vi "Save Packets.vi"(5 "Save Format":u16, 6 "Headers":string[](array[string]), 7 "Path":path, 8 "error in":errorcluster, 9 "SAVE TO CSV":refnum<vi>, 10 "Packets":refnum<vi>, 11 "Interface Name String":string) -> (0 "error out":errorcluster, 3 "Status Message":string)   [LabVIEW 2025, in "Automotive Ethernet Bus Monitor UI.lvlib"]
doc: "Save the current Package Table to a file."
uses:
  Automotive Ethernet Bus Monitor UI.lvlib
  <vilib>/Utility/file.llb/Write Delimited Spreadsheet (string).vi
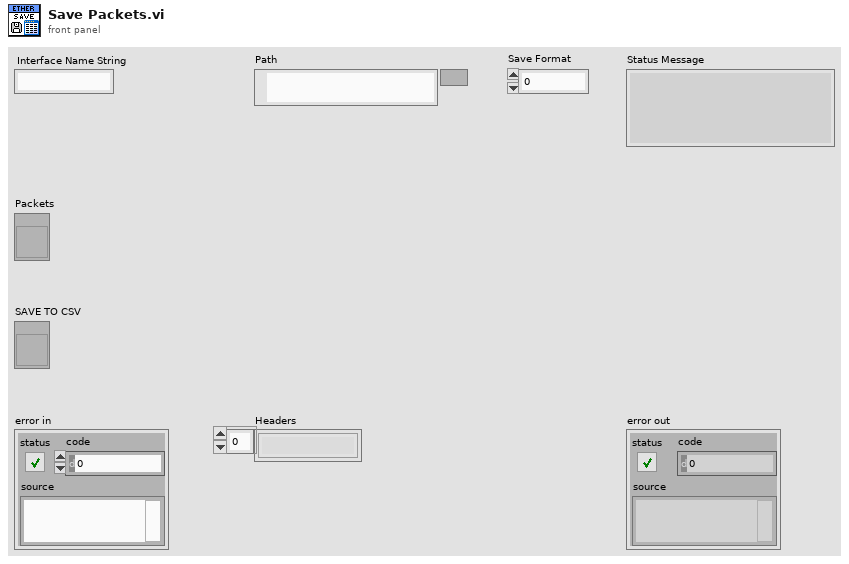
[diagram p1: front panel]
types:
  T1 = enum16{"open", "open or create", "create or replace", "create", "open (read-only)"}
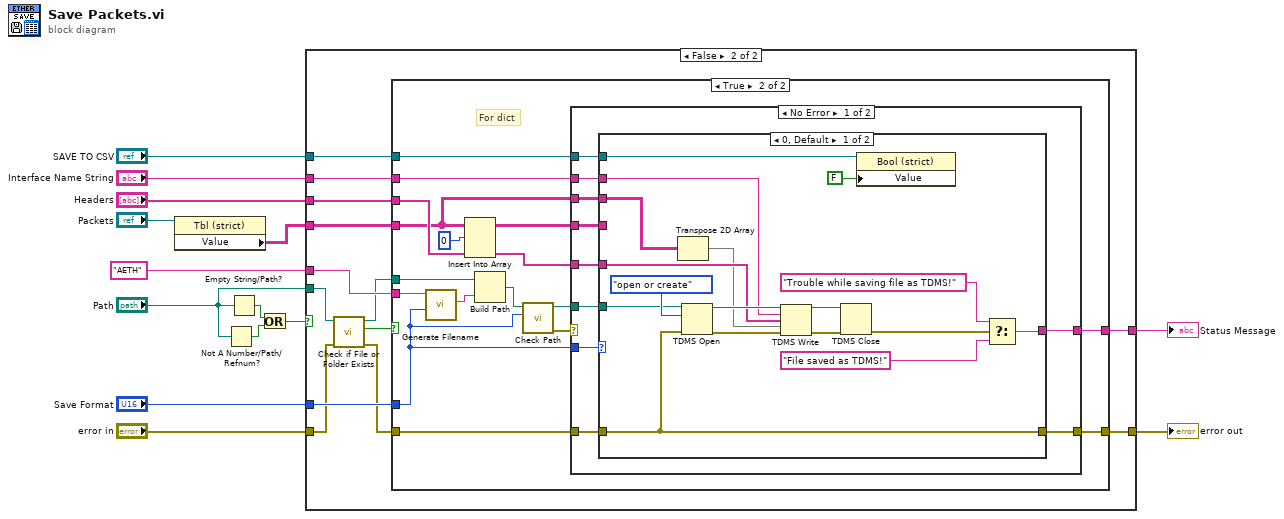
[diagram p0: block diagram]
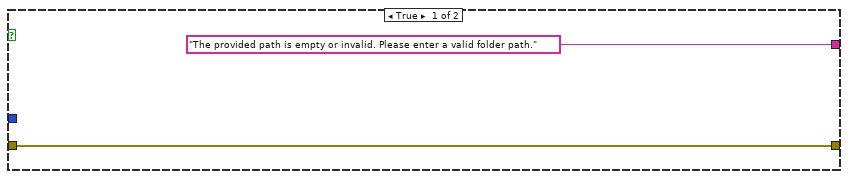
[diagram p2: hidden frame]
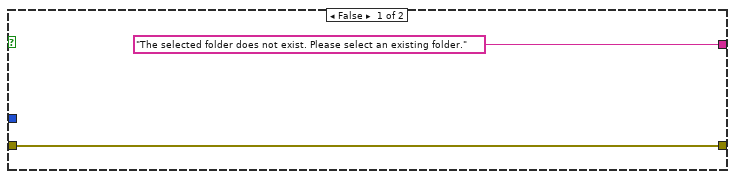
[diagram p3: hidden frame]
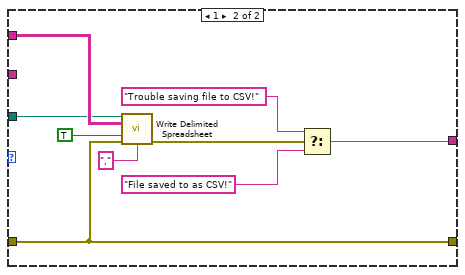
[diagram p4: hidden frame]
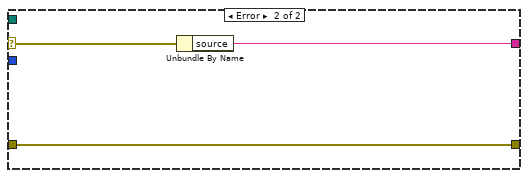
[diagram p5: hidden frame]
diagram:
  n1 = property class="Tbl (strict)"(reference="Packets") -> ("Value"=w5:string[][])  [unwired: 1 in, 2 out]
  n2 = Not A Number/Path/Refnum?(number/path/refnum="Path") -> (NaN/Path/Refnum?=w13:bool)
  n3 = Empty String/Path?(string/path="Path") -> (empty?=w12:bool)
  n4 = Or(x=w12, y=w13) -> (x .or. y?=w14:bool)
  n5 = case shown="False" w14 {
    tunnel: [w15 w29] -> w7
    tunnel: "Headers" -> [_ w28]
    tunnel: w5 -> [_ w27]
    tunnel: "error in" -> [w15 w19]
    tunnel: "Save Format" -> [_ w25]
    tunnel: "AETH" ("bustype in") -> [_ w24]
    tunnel: "Path" -> [_ w23]
    tunnel: ["The provided path is empty or invalid. Please enter a valid folder path." ("source") w21] -> w11
    tunnel: "Interface Name String" -> [_ w18]
    tunnel: "SAVE TO CSV" -> [_ w17]
    frame True {
    }
    frame False {
      n6 = call <vilib>:"Check if File or Folder Exists.vi"("error in (no error)"=w19, "path"=w23) -> ("error out"=w20:errorcluster, "file or folder exists?"=w26:bool, "dup path"=w22:path)  [unwired: 7 in]
      n7 = case shown="True" w26 {
        tunnel: [w31 w45] -> w29
        tunnel: w28 -> [_ w44]
        tunnel: w27 -> [_ w43]
        tunnel: w20 -> [w31 w38]
        tunnel: w22 -> [_ w37]
        tunnel: w25 -> [_ w36]
        tunnel: w24 -> [_ w35]
        tunnel: ["The selected folder does not exist. Please select an existing folder." ("source") w34] -> w21
        tunnel: w18 -> [_ w33]
        tunnel: w17 -> [_ w32]
        frame False {
        }
        frame True {
          # "For dict"
          n8 = call "Generate Filename.vi"("format  in"=w36, "bustype in"=w35) -> ("filename"=w39:string)  [unwired: 9 in]
          n9 = Insert Into Array(array=w43, index (row)=0, new element=w44) -> (w46:string[][])  [unwired: 1 in]
          n10 = Build Path(base path=w37, name or relative path=w39) -> (appended path=w40:path)
          n11 = call "Check Path.vi"("SAVE TYPE"=w36, "file in"=w40) -> ("Error Out"=w41:errorcluster, "path"=w42:path)  [unwired: 8 in]
          n12 = case shown="No Error" w41 {
            selector: w41 -> [_ w86]
            tunnel: w46 -> [w57 _]
            tunnel: w38 -> [w56 w85]
            tunnel: [w55 w85] -> w45
            tunnel: w44 -> [w54 _]
            tunnel: w43 -> [w53 _]
            tunnel: w42 -> [w52 _]
            tunnel: w36 -> [w51 _]
            tunnel: [w50 w84] -> w34
            tunnel: w33 -> [w49 _]
            tunnel: w32 -> [w48 _]
            frame No Error {
              n13 = case shown="0, Default" w51 {
                tunnel: w57 -> [_ w83]
                tunnel: w56 -> [w62 w76]
                tunnel: w52 -> [w68 w79]
                tunnel: [w62 w76] -> w55
                tunnel: w54 -> [w69 _]
                tunnel: w53 -> [w64 _]
                tunnel: [w61 w75] -> w50
                tunnel: w49 -> [w59 _]
                tunnel: w48 -> [w58 _]
                frame 0, Default {
                  n14 = Transpose 2D Array(2D array=w64) -> (transposed array=w66:string[][])
                  n15 = TDMS Open(8:w62, 10:T1."open or create" ("operation (0:open)"), 11:w68) -> (0:w72:errorcluster, 3:w73:refnum<k34>)  [unwired: 4 in]
                  n16 = TDMS Write(0:w73, 5:w59, 7:w69, 9:w66, 11:w72) -> (4:w70:refnum<k34>, 15:w71:errorcluster)  [unwired: 1 in, 2 out]
                  n17 = TDMS Close(8:w71, 11:w70) -> (0:w60:errorcluster)  [unwired: 1 out]
                  n18 = property class="Bool (strict)"(reference=w58, "Value"=FALSE) -> ()  [unwired: 1 in, 2 out]
                  n19 = Select(t="Trouble while saving file as TDMS!" ("f"), s=w60, f="File saved as TDMS!") -> (s? t:f=w61:string)
                }
                frame 1 {
                  n20 = call-poly <vilib>:"Write Delimited Spreadsheet.vi"("file path (dialog if empty)"=w79, "2D data"=w83, "append to file? (new file:F)"=TRUE, "error in (no error)"=w76, "delimiter (\\t)"="," ("delimiter (\\t)")) -> ("error out"=w78:errorcluster)  [unwired: 9 in, 1 out]
                  n21 = Select(t="Trouble saving file to CSV!" ("f"), s=w78, f="File saved to as CSV!") -> (s? t:f=w75:string)
                }
              }
            }
            frame Error {
              n22 = Unbundle By Name(w86) -> ("source"=w84:string)
            }
          }
        }
      }
    }
  }
  "error out" <- w7
  "Status Message" <- w11
